vi "Day 24.vi"() -> ()   [LabVIEW 2021]
panel:
  out "Minimum Model Number":string
  out "Maximum Model Number":string
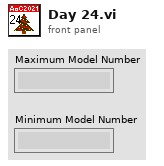
[diagram p1: front panel]
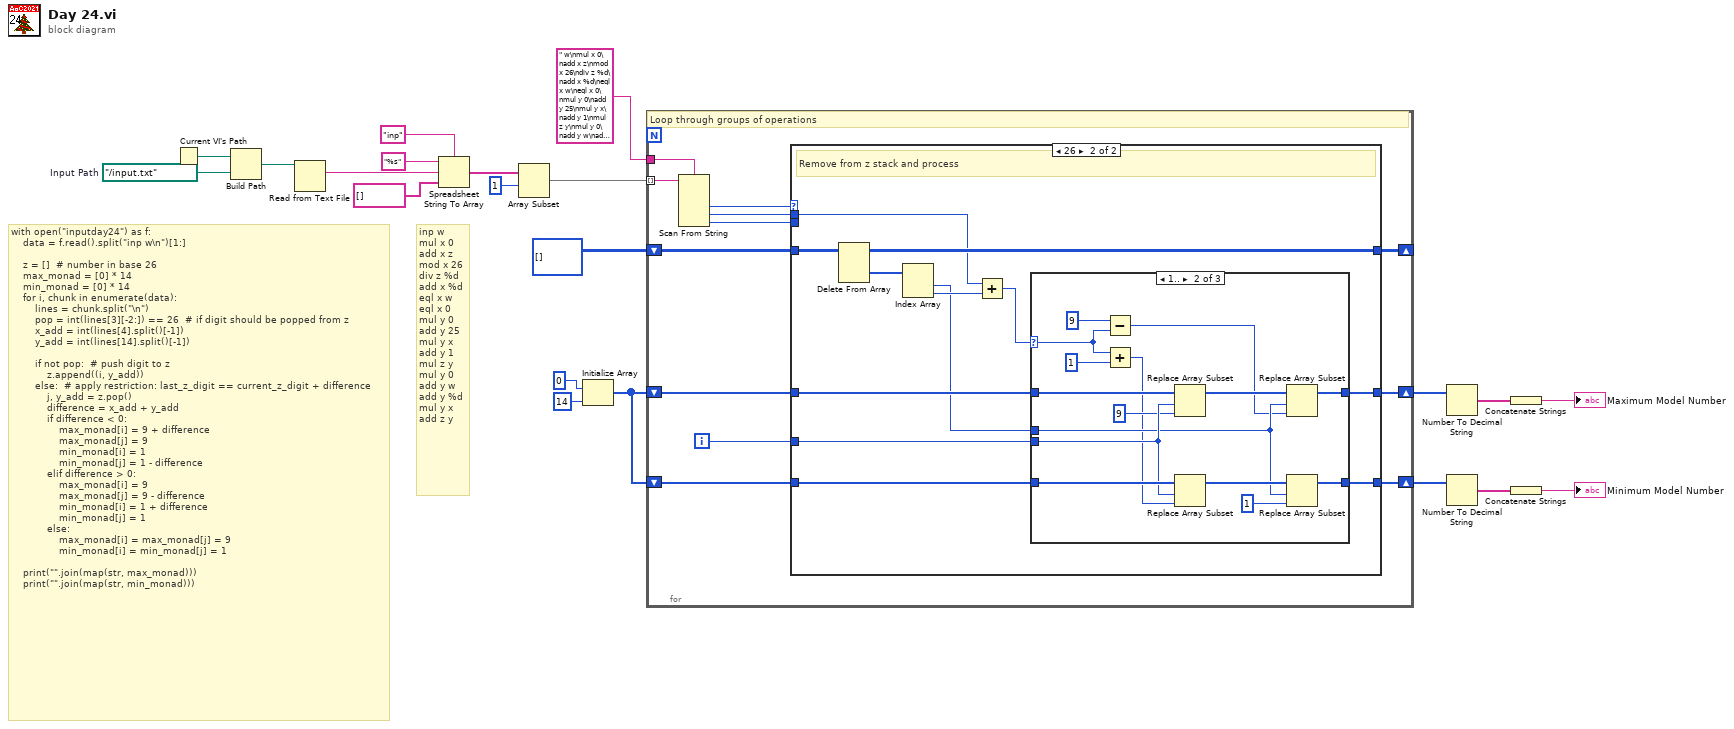
[diagram p0: block diagram]
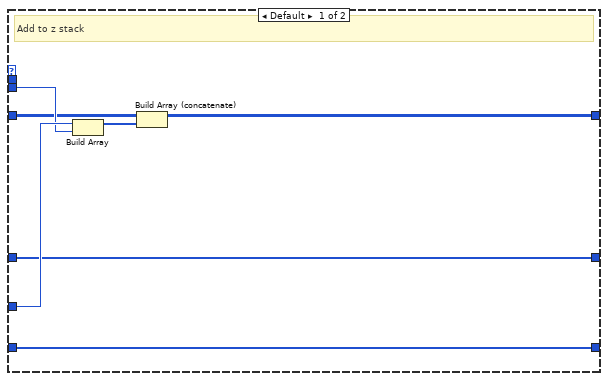
[diagram p2: hidden frame]
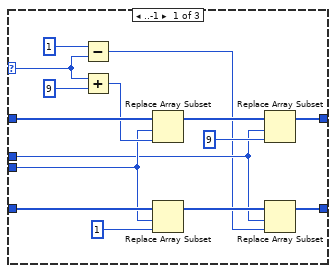
[diagram p3: hidden frame]
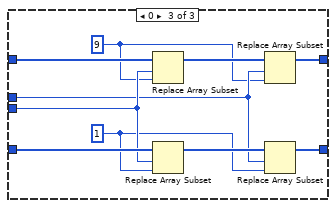
[diagram p4: hidden frame]
diagram:
  w21 = path "../input.txt"  # Input Path
  # "inp w\nmul x 0\nadd x z\nmod x 26\ndiv z %d\nadd x %d\neql x w\neql x 0\nmul y 0\nadd y 25\nmul y x\nadd y 1\nmul z y\nmul y 0\nadd y w\nadd y %d\nmul y x\nadd z y"
  # "with open(\"inputday24\") as f:\n    data = f.read().split(\"inp w\\n\")[1:]\n\n    z = []  # number in base 26\n    max_monad = [0] * 14\n    min_monad = [0] * 14\n    for i, chunk in enumerate(data):\n        lines = chunk.split(\"\\n\")\n        pop = int(lines[3][-2:]) == 26  # if digit should be popped from z\n        x_add = int(lines[4].split()[-1])\n        y_add = int(lines[14].split()[-1])\n\n        if not pop:  # push digit to z\n            z.append((i, y_add))\n        else:  # apply restriction: last_z_digit == current_z_digit + difference\n            j, y_add = z.pop()\n            difference = x_add + y_add\n            if difference < 0:\n                max_monad[i] = 9 + difference\n                max_monad[j] = 9\n                min_monad[i] = 1\n                min_monad[j] = 1 - difference\n            elif difference > 0:\n                max_monad[i] = 9\n                max_monad[j] = 9 - difference\n                min_monad[i] = 1 + difference\n                min_monad[j] = 1\n            else:\n                max_monad[i] = max_monad[j] = 9\n                min_monad[i] = min_monad[j] = 1\n\n    print(\"\".join(map(str, max_monad)))\n    print(\"\".join(map(str, min_monad)))"
  n1 = Current VI's Path() -> (path=w20:path)
  n2 = Build Path(base path=w20, name or relative path=w21) -> (appended path=w19:path)
  n3 = Read from Text File(file (use dialog)=w19) -> (text=w18:string)  [unwired: 3 in, 3 out]
  n4 = Spreadsheet String To Array(delimiter (Tab)="inp", format string="%s", spreadsheet string=w18, array type (2D Dbl)=string[] []) -> (array=w14:string[])
  n5 = Array Subset(array=w14, index=1) -> (w1:string[])  [unwired: 1 in]
  n6 = Initialize Array(0, 14) -> (w10:i32[])
  n7 = for {
    shift-right: [w32] -> w8
    shift-left: w10 -> [w31]
    shift-right: [w30] -> w7
    shift-left: w10 -> [w29]
    shift-right: [w33] -> _
    shift-left: i32[][] [] -> [w22]
    tunnel: " w\nmul x 0\nadd x z\nmod x 26\ndiv z %d\nadd x %d\neql x w\neql x 0\nmul y 0\nadd y 25\nmul y x\nadd y 1\nmul z y\nmul y 0\nadd y w\nadd y %d\nmul y x\nadd z y" -> [w24]
    tunnel: w1 -> [w23] mode=indexing
    i -> [w28]
    # "Loop through groups of operations"
    n8 = Scan From String(format string=w24, input string=w23) -> (output 1=w27:i32, output 2=w26:i32, output 3=w25:i32)  [unwired: 5 in, 3 out]
    n9 = case shown="26" w27 {
      tunnel: w26 -> [_ w49]
      tunnel: w25 -> [w39 _]
      tunnel: w22 -> [w38 w52]
      tunnel: w28 -> [w40 w42]
      tunnel: [w36 w51] -> w33
      tunnel: [w35 w46] -> w32
      tunnel: w31 -> [w35 w45]
      tunnel: [w34 w44] -> w30
      tunnel: w29 -> [w34 w43]
      frame Default {
        # "Add to z stack"
        n10 = Build Array(w40, w39) -> (w37:i32[])
        n11 = Build Array (concatenate)(w38, w37) -> (w36:i32[][])
      }
      frame 26 {
        # "Remove from z stack and process"
        n12 = Delete From Array(array=w52) -> (deleted portion=w50:i32[], array with subset deleted=w51:i32[][])  [unwired: 3 in]
        n13 = Index Array(array=w50) -> (element #1=w41:i32, element #2=w48:i32)  [unwired: 2 in]
        n14 = Add(x=w49, y=w48) -> (x+y=w47:i32)
        n15 = case shown="1.." w47 {
          selector: w47 -> [w58 w76 _]
          tunnel: [w63 w79 w90] -> w46
          tunnel: w45 -> [w67 w82 w92]
          tunnel: [w53 w72 w85] -> w44
          tunnel: w43 -> [w61 w78 w89]
          tunnel: w42 -> [w60 w77 w88]
          tunnel: w41 -> [w56 w74 w86]
          frame ..-1 {
            n16 = Subtract(x=1, y=w58) -> (x-y=w54:i32)
            n17 = Add(x=w58, y=9) -> (x+y=w65:i32)
            n18 = Replace Array Subset(array=w67, new element=w65, index=w60) -> (w64:i32[])
            n19 = Replace Array Subset(array=w61, new element=1 ("new element/subarray"), index=w60) -> (w57:i32[])
            n20 = Replace Array Subset(array=w64, new element=9 ("new element/subarray"), index=w56) -> (w63:i32[])
            n21 = Replace Array Subset(array=w57, new element=w54, index=w56) -> (w53:i32[])
          }
          frame 1.. {
            n22 = Subtract(x=9 ("y"), y=w76) -> (x-y=w70:i32)
            n23 = Add(x=w76, y=1 ("x")) -> (x+y=w69:i32)
            n24 = Replace Array Subset(array=w82, new element=9 ("new element/subarray"), index=w77) -> (w80:i32[])
            n25 = Replace Array Subset(array=w78, new element=w69, index=w77) -> (w75:i32[])
            n26 = Replace Array Subset(array=w80, new element=w70, index=w74) -> (w79:i32[])
            n27 = Replace Array Subset(array=w75, new element=1 ("new element/subarray"), index=w74) -> (w72:i32[])
          }
          frame 0 {
            w83 = 1 ("new element/subarray")
            w84 = 9 ("new element/subarray")
            n28 = Replace Array Subset(array=w92, new element=w84, index=w88) -> (w91:i32[])
            n29 = Replace Array Subset(array=w89, new element=w83, index=w88) -> (w87:i32[])
            n30 = Replace Array Subset(array=w91, new element=w84, index=w86) -> (w90:i32[])
            n31 = Replace Array Subset(array=w87, new element=w83, index=w86) -> (w85:i32[])
          }
        }
      }
    }
  }
  n32 = Number To Decimal String(number=w8) -> (decimal integer string=w6:string[])  [unwired: 1 in]
  n33 = Number To Decimal String(number=w7) -> (decimal integer string=w3:string[])  [unwired: 1 in]
  n34 = Concatenate Strings(w6) -> (→"Maximum Model Number":string)
  n35 = Concatenate Strings(w3) -> (→"Minimum Model Number":string)
